vi "Spectral mode.vi"() -> ()   [LabVIEW 2018]
panel:
  in  "Constante de condition\n(Voir l'aide contextuelle)":bool
  out "Data":i32[][](graph)
  out "trigAddress":i32
  in  "Commande tab":T1(tab)
  in  "Area Number to Display":i32
  in  "Reformat":bool
  in  "GAIN":u16(ring) caption="Device Name" items=["High Light", "Best Dynamic Range", "High Sensitivity"]
  in  "ADC":u16(ring) caption="Device Name" items=["20 kHz       ", " 1 MHz       ", "500 kHz Wrap"]
  in  "Number of Areas :":u16=1 min=1 step=1
  in  "Integration time (ms) :":i16=10
  out "Uniques ID":u16(ring) items=["CCD1", "CCD2"]
  in  "Device Name":u16(ring) items=["Synapse CCD (Lateral)", "Synapse_IGA (Axial)"]
  in  "Signal type :":enum16{"TTL Rising Edge", "TTL Falling Edge"}(ring)=enum."TTL Falling Edge"
  in  "Trigger Type :":u16(ring) items=["On Start"=1, "Per Acquisition"=2]
  in  "trigSigTypeString":string
  in  "trigEventString":string
  in  "Enable InputTriggers :":bool
  in  "Number of Cleans":i32=1
  in  "MultiAcqShutterMode":i32(ring)=3 items=["Open For All Spectra"=1, "Open for Each Spectrum"=3]
  in  "Accumulations:":u16=10 min=1 step=1
  in  "Multi Accumulation mode:":bool
  out "Y Pixels:":i32=256
  out "DataSize":i32=1024
  out "X Pixels:":i32=1024
  out "Firmware\nVersion":string="V1.20 CCD_4000"
  out "Acq Time(ms)":u32=3401
  out "Gain Number":i32[](array[numeric])=[10, 11, 12, 13, 8, 2]
  out "ADC Number":i32[](array[numeric])=[0, 1, 2, 3, 4]
  in  "save":bool
  out "initialized ?":bool=TRUE
  in  "Continuous":bool
  in  "CCD Busy":bool
  in  "ShutterOpen":bool=TRUE caption="Shutter enable"
  out "temp graph":dbl(graph)=-134.538067
  in  "Temperature":bool
  out "areas :":i32[][](array[numeric])=[[1], [1], [1], [1024], [256], [1], [256]]
  in  "Acquire":bool
  in  "Setup":bool
  in  "Close":bool=TRUE
  out "indicator":string="Ready !"
  in  "initialize":bool
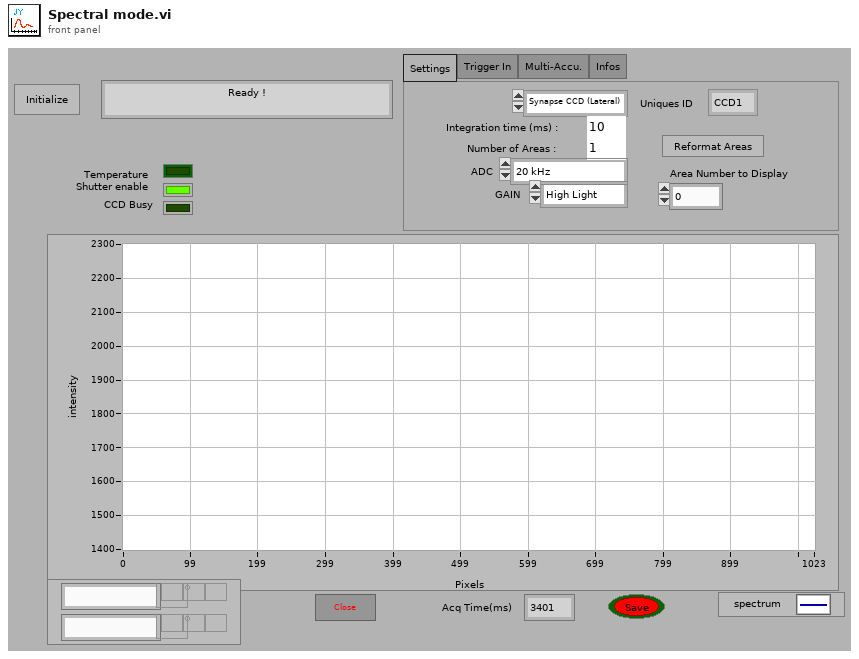
[diagram p1: front panel]
types:
  T1 = enum32{"Settings", "Trigger In", "Multi-Accu.", "Infos"}
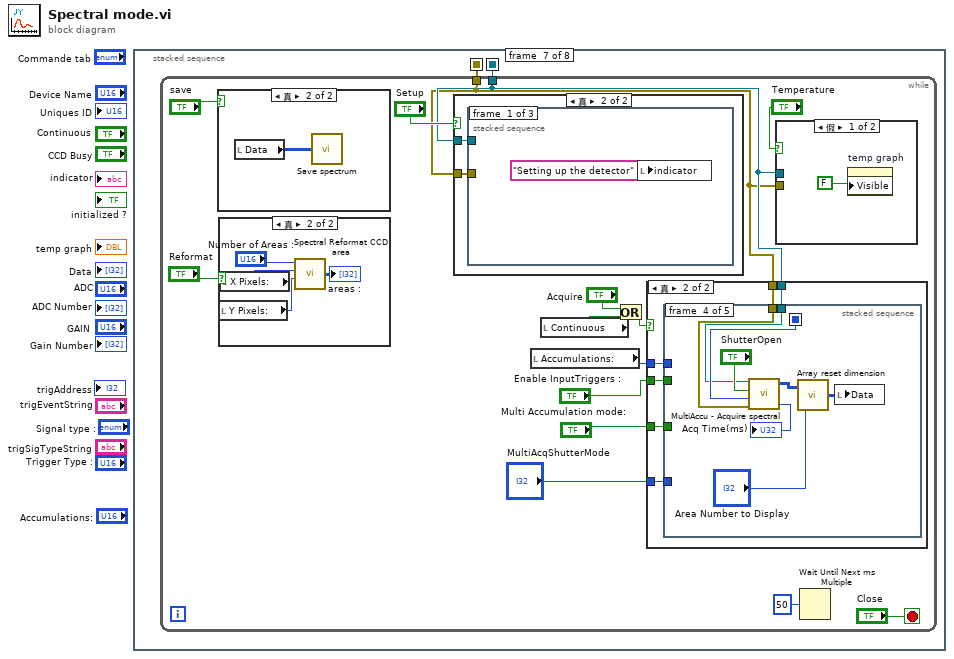
[diagram p0: block diagram]
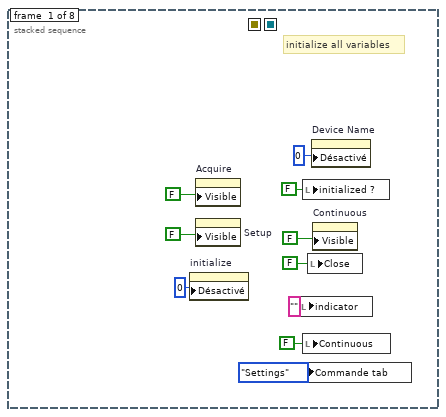
[diagram p2: hidden frame]
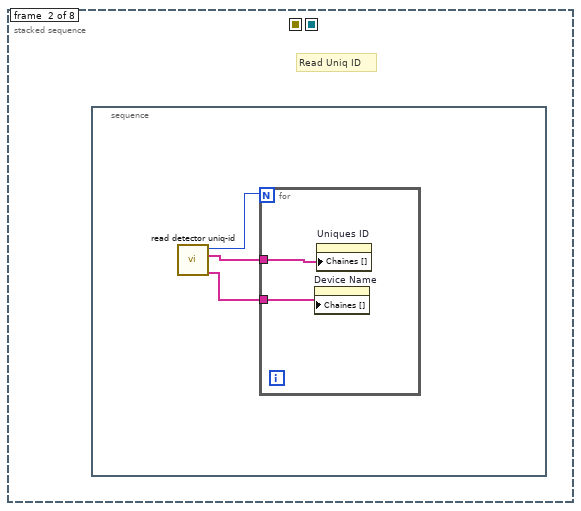
[diagram p3: hidden frame]
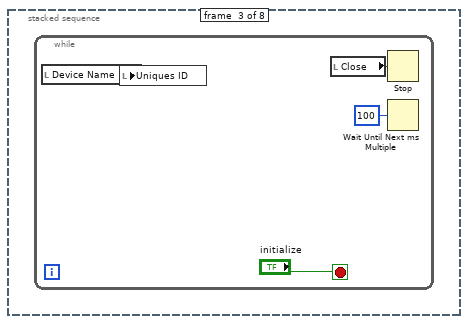
[diagram p4: hidden frame]
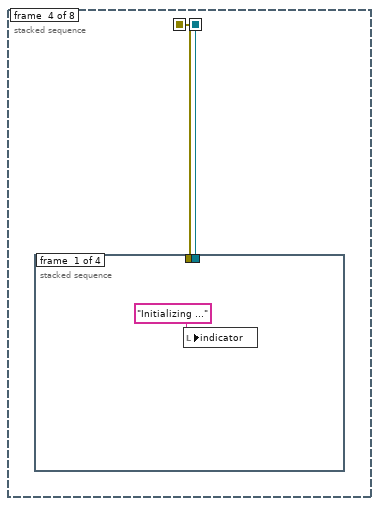
[diagram p5: hidden frame]
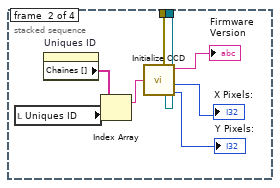
[diagram p6: hidden frame]
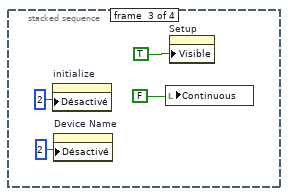
[diagram p7: hidden frame]
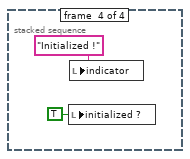
[diagram p8: hidden frame]
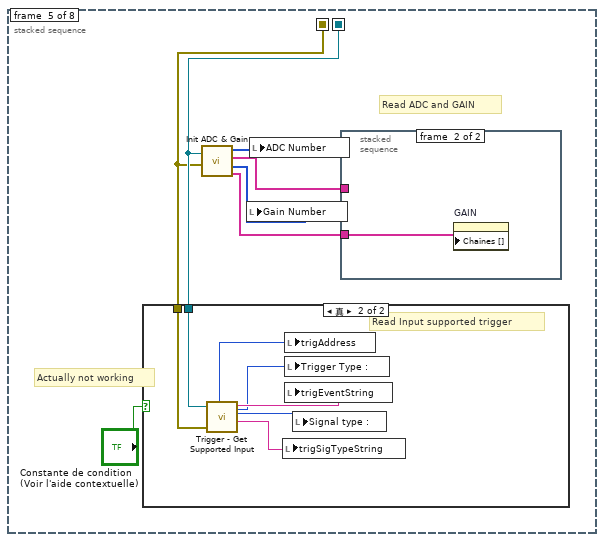
[diagram p9: hidden frame]
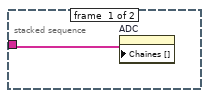
[diagram p11: hidden frame]
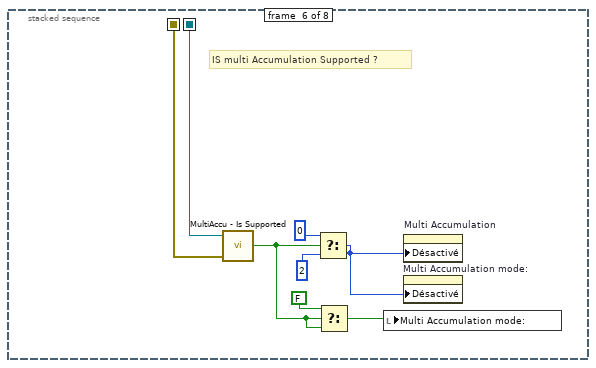
[diagram p12: hidden frame]
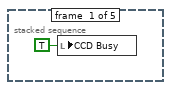
[diagram p15: hidden frame]
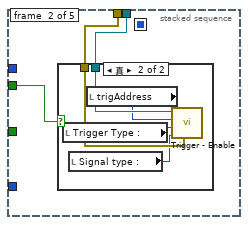
[diagram p16: hidden frame]
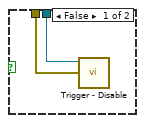
[diagram p17: hidden frame]
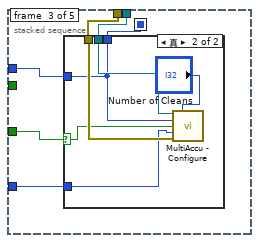
[diagram p18: hidden frame]
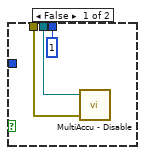
[diagram p19: hidden frame]
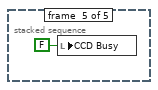
[diagram p20: hidden frame]
diagram:
  n1 = stacked-sequence {
    seq-local: [_ _ _ w21 _ _ _ _] -> [_ _ _ _ w39 w59 w62 w150]
    seq-local: [_ _ _ w20 _ _ _ _] -> [_ _ _ _ w40 w60 w61 w151]
    frame #0 {
      # "initialize all variables"
      n2 = property on="initialize" class="Bool"("Désactivé"=u8 0) -> ()  [unwired: 2 in, 2 out]
      n3 = property on="Acquire" class="Bool"("Visible"=FALSE) -> ()  [unwired: 2 in, 2 out]
      n4 = property on="Setup" class="Bool"("Visible"=FALSE) -> ()  [unwired: 2 in, 2 out]
      n5 = local write "indicator"("" ("indicator")) -> ()
      n6 = local write "Commande tab"(T1."Settings" ("Commande tab")) -> ()
      n7 = local write "initialized ?"(FALSE ("initialized ?")) -> ()
      n8 = local write "Continuous"(FALSE ("Continuous")) -> ()
      n9 = local write "Close"(FALSE ("Close")) -> ()
      n10 = property on="Device Name" class="Ring (严格)"("Désactivé"=u8 0) -> ()  [unwired: 2 in, 2 out]
      n11 = property on="Continuous" class="Bool (严格)"("Visible"=FALSE) -> ()  [unwired: 2 in, 2 out]
    }
    frame #1 {
      # "Read Uniq ID"
      n12 = stacked-sequence {
        frame #0 {
          n13 = call <userlib>:"read detector uniq-id.vi"() -> ("nbr of components"=w13:i32, "UniqueID"=w12:string[], "Name"=w11:string[])  [unwired: 4 out]
          n14 = for {
            N: w13 -> [_]
            tunnel: w12 -> [w15]
            tunnel: w11 -> [w14]
            n15 = property on="Device Name" class="Ring (严格)"("Chaînes []"=w14) -> ()  [unwired: 2 in, 2 out]
            n16 = property on="Uniques ID" class="Ring (严格)"("Chaînes []"=w15) -> ()  [unwired: 2 in, 2 out]
          }
        }
      }
    }
    frame #2 {
      n17 = while {
        stop <- "initialize" stop-if-true
        n18 = local read "Device Name"() -> (w18:u16)
        n19 = local write "Uniques ID"(w18) -> ()
        n20 = local read "Close"() -> (w16:bool)
        n21 = Stop(stop? (T)=w16) -> ()
        n22 = Wait Until Next ms Multiple(millisecond multiple=u32 100 ("n millisecondes")) -> ()  [unwired: 1 out]
      }
    }
    frame #3 {
      n23 = stacked-sequence {
        tunnel: [_ w28 _ _] -> w21
        tunnel: [_ w27 _ _] -> w20
        frame #0 {
          n24 = local write "indicator"("Initializing ..." ("indicator")) -> ()
        }
        frame #1 {
          n25 = local read "Uniques ID"() -> (w25:u16)
          n26 = property on="Uniques ID" class="Ring (严格)"() -> ("Chaînes []"=w26:string[])  [unwired: 2 in, 2 out]
          n27 = Index Array(array=w26, index=w25) -> (element=w24:string)
          n28 = call <userlib>:"Initialize CCD.vi"("Unique id:"=w24) -> ("activeYPixels"=→"Y Pixels:":i32, "JYCCDLib.IJYCCDReqd"=w27:refnum<k7>, "activeXPixels"=→"X Pixels:":i32, "sortie d'erreur"=w28:errorcluster, "FirmwareVersion"=→"Firmware\nVersion":string)  [unwired: 3 out]
        }
        frame #2 {
          n29 = property on="initialize" class="Bool"("Désactivé"=u8 2) -> ()  [unwired: 2 in, 2 out]
          n30 = property on="Device Name" class="Ring (严格)"("Désactivé"=u8 2) -> ()  [unwired: 2 in, 2 out]
          n31 = local write "Continuous"(FALSE ("Continuous")) -> ()
          n32 = property on="Setup" class="Bool"("Visible"=TRUE) -> ()  [unwired: 2 in, 2 out]
        }
        frame #3 {
          n33 = local write "initialized ?"(TRUE ("initialized ?")) -> ()
          n34 = local write "indicator"("Initialized !" ("indicator")) -> ()
        }
      }
    }
    frame #4 {
      # "Actually not working"
      # "Read ADC and GAIN"
      n35 = case shown="真" "Constante de condition\n(Voir l'aide contextuelle)" {
        tunnel: w40 -> [_ w50]
        tunnel: w39 -> [_ w49]
        frame False {
        }
        frame True {
          # "Read Input supported trigger"
          n36 = call <userlib>:"Trigger - Get Supported Input.vi"("JYCCDLib.IJYCCDReqd"=w50, "Error Input"=w49) -> ("trigAddress"=w44:i32, "eventPtr"=w45:i32, "trigEventString"=w48:string, "trigSigType"=w47:i32, "trigSigTypeString"=w46:string)  [unwired: 4 out]
          n37 = local write "trigSigTypeString"(w46) -> ()
          n38 = local write "trigAddress"(w44) -> ()
          n39 = local write "Trigger Type :"(w45) -> ()
          n40 = local write "trigEventString"(w48) -> ()
          n41 = local write "Signal type :"(w47) -> ()
        }
      }
      n42 = call <userlib>:"Init ADC & Gain.vi"("JYCCDLib.IJYCCDReqd"=w40, "input error"=w39) -> ("ADC Number"=w38:i32[], "ADC description"=w43:string[], "Gain Number"=w41:i32[], "Gain description"=w42:string[])
      n43 = local write "Gain Number"(w41) -> ()
      n44 = local write "ADC Number"(w38) -> ()
      n45 = stacked-sequence {
        tunnel: w43 -> [w51 _]
        tunnel: w42 -> [_ w52]
        frame #0 {
          n46 = property on="ADC" class="Ring (严格)"("Chaînes []"=w51) -> ()  [unwired: 2 in, 2 out]
        }
        frame #1 {
          n47 = property on="GAIN" class="Ring (严格)"("Chaînes []"=w52) -> ()  [unwired: 2 in, 2 out]
        }
      }
    }
    frame #5 {
      # "IS multi Accumulation Supported ?"
      n48 = call <userlib>:"MultiAccu - Is Supported.vi"("Error In"=w59, "JYCCDLib.IJYCCDReqd"=w60) -> ("IsOperatingModeSupported"=w53:bool)  [unwired: 3 out]
      n49 = Select(t=0, s=w53, f=2) -> (s? t:f=w56:i32)
      n50 = Select(t=FALSE, s=w53, f=w53) -> (s? t:f=w55:bool)
      n51 = local write "Multi Accumulation mode:"(w55) -> ()
      n52 = property on="Multi Accumulation" class="Bool (严格)"("Désactivé"=w56) -> ()  [unwired: 2 in, 2 out]
      n53 = property on="Multi Accumulation mode:" class="Bool (严格)"("Désactivé"=w56) -> ()  [unwired: 2 in, 2 out]
    }
    frame #6 {
      n54 = while {
        tunnel: w61 -> [w70]
        tunnel: w62 -> [w68]
        stop <- "Close" stop-if-true
        n55 = case shown="真" "save" {
          frame False {
          }
          frame True {
            n56 = local read "Data"() -> (w78:i32[][])
            n57 = call "Save spectrum.vi"("Datas 2"=w78) -> ()  [unwired: 1 out]
          }
        }
        n58 = case shown="真" "Reformat" {
          frame False {
          }
          frame True {
            n59 = local read "Y Pixels:"() -> (w128:i32)
            n60 = local read "X Pixels:"() -> (w130:i32)
            n61 = call <userlib>:"Spectral Reformat CCD area.vi"("Y Pixels:"=w128, "X Pixels:"=w130, "numAreas"="Number of Areas :") -> ("areas :"=→"areas :":i32[][])  [unwired: 3 out]
          }
        }
        n62 = case shown="真" "Setup" {
          tunnel: w68 -> [_ w133]
          tunnel: w70 -> [_ w132]
          frame False {
          }
          frame True {
            n63 = stacked-sequence {
              tunnel: w133 -> [_ w147 _]
              tunnel: w132 -> [_ w144 _]
              frame #0 {
                n64 = local write "indicator"("Setting up the detector" ("indicator")) -> ()
              }
              frame #1 {
                w145 = 1 items=["JYMCD_ACQ_FORMAT_IMAGE", "JYMCD_ACQ_FORMAT_SCAN"] ("Acquisition type")
                n65 = local read "Gain Number"() -> (w139:i32[])
                n66 = local read "GAIN"() -> (w135:u16)
                n67 = local read "ADC Number"() -> (w140:i32[])
                n68 = local read "ADC"() -> (w136:u16)
                n69 = Index Array(array=w139, index=w135) -> (element=w137:i32)
                n70 = Index Array(array=w140, index=w136) -> (element=w138:i32)
                n71 = local read "Number of Areas :"() -> (w142:u16)
                n72 = local read "areas :"() -> (w143:i32[][])
                n73 = call <userlib>:"Setup CCD.vi"("numAreas"=w142, "areas :"=w143, "JYCCDLib.IJYCCDReqd"=w144, "entrée d'erreur (pas d'erreur)"=w147, "Acquisition type"=w145, "Gain"=w137, "Select ADC"=w138, "Integration time(ms)"="Integration time (ms) :") -> ("DataSize"=→"DataSize":i32)  [unwired: 1 out]
              }
              frame #2 {
                w148 = TRUE ("Visible")
                n74 = property on="Continuous" class="Bool (严格)"("Visible"=w148) -> ()  [unwired: 2 in, 2 out]
                n75 = property on="Acquire" class="Bool"("Visible"=w148) -> ()  [unwired: 2 in, 2 out]
                n76 = local write "indicator"("Ready !" ("indicator")) -> ()
              }
            }
          }
        }
        n77 = local read "Accumulations:"() -> (w65:u16)
        n78 = local read "Continuous"() -> (w71:bool)
        n79 = Or(x="Acquire", y=w71) -> (x .or. y?=w67:bool)
        n80 = case shown="真" w67 {
          tunnel: w70 -> [_ w84]
          tunnel: w68 -> [_ w83]
          tunnel: "Enable InputTriggers :" -> [_ w82]
          tunnel: "Multi Accumulation mode:" -> [_ w81]
          tunnel: w65 -> [_ w80]
          tunnel: "MultiAcqShutterMode" -> [_ w79]
          frame False {
          }
          frame True {
            n81 = stacked-sequence {
              seq-local: [_ _ w97 _ _] -> [_ _ _ w116 _]
              tunnel: w84 -> [_ w86 w101 w115 _]
              tunnel: w83 -> [_ w87 w100 w114 _]
              tunnel: w82 -> [_ w88 _ _ _]
              tunnel: w81 -> [_ _ w99 _ _]
              tunnel: w80 -> [_ _ w98 _ _]
              tunnel: w79 -> [_ _ w96 _ _]
              frame #0 {
                n82 = local write "CCD Busy"(TRUE ("CCD Busy")) -> ()
              }
              frame #1 {
                n83 = case shown="真" w88 {
                  tunnel: w87 -> [w89 w95]
                  tunnel: w86 -> [w90 w94]
                  frame False {
                    n84 = call <userlib>:"Trigger - Disable.vi"("Error In"=w89, "JYCCDLib.IJYCCDReqd"=w90) -> ()  [unwired: 6 out]
                  }
                  frame True {
                    n85 = local read "Trigger Type :"() -> (w91:u16)
                    n86 = local read "Signal type :"() -> (w92:enum16{"TTL Rising Edge", "TTL Falling Edge"})
                    n87 = local read "trigAddress"() -> (w93:i32)
                    n88 = call <userlib>:"Trigger - Enable.vi"("Error In"=w95, "sigType"=w92, "event"=w91, "trigAddress"=w93, "JYCCDLib.IJYCCDReqd"=w94) -> ()  [unwired: 3 out]
                  }
                }
              }
              frame #2 {
                n89 = case shown="真" w99 {
                  selector: w99 -> [_ w107]
                  tunnel: w101 -> [w104 w110]
                  tunnel: w100 -> [w103 w109]
                  tunnel: w98 -> [_ w108]
                  tunnel: [u16 1 ("Accumulations:") w108] -> w97
                  tunnel: w96 -> [_ w106]
                  frame False {
                    n90 = call <userlib>:"MultiAccu - Disable.vi"("Error In"=w103, "JYCCDLib.IJYCCDReqd"=w104) -> ()  [unwired: 4 out]
                  }
                  frame True {
                    n91 = call <userlib>:"MultiAccu - Configure.vi"("JYCCDLib.IJYCCDReqd"=w110, "Cleans Before"="Number of Cleans", "Accumulations:"=w108, "MultiAcqHardwareMode"=w107, "MultiAcqShutterMode"=w106, "Error In"=w109) -> ()  [unwired: 1 in, 9 out]
                  }
                }
              }
              frame #3 {
                n92 = call <userlib>:"MultiAccu - Acquire spectral.vi"("error in"=w114, "Accumulations:"=w116, "ShutterOpen"="ShutterOpen", "JYCCDLib.IJYCCDReqd"=w115) -> ("Acq Time(ms)"=→"Acq Time(ms)":u32, "Array Out"=w113:i32[][][])  [unwired: 1 out]
                n93 = call <userlib>:"Array reset dimension.vi"("Area Number"="Area Number to Display", "Array In"=w113) -> ("Array Out"=w112:i32[][])
                n94 = local write "Data"(w112) -> ()
              }
              frame #4 {
                n95 = local write "CCD Busy"(FALSE ("CCD Busy")) -> ()
              }
            }
          }
        }
        n96 = case shown="假" "Temperature" {
          tunnel: w70 -> [_ w122]
          tunnel: w68 -> [_ w121]
          frame False {
            n97 = property on="temp graph" class="WFChart (严格)"("Visible"=FALSE) -> ()  [unwired: 2 in, 2 out]
          }
          frame True {
            n98 = stacked-sequence {
              tunnel: w122 -> [_ w127]
              tunnel: w121 -> [_ w126]
              frame #0 {
                n99 = property on="temp graph" class="WFChart (严格)"("Visible"=TRUE) -> ()  [unwired: 2 in, 2 out]
              }
              frame #1 {
                w125 = u16 0 items=["° Celsius", "Kelvin", "° Farenheit"] ("units")
                n100 = call <userlib>:"read temperature.vi"("entrée d'erreur (pas d'erreur)"=w126, "units"=w125, "JYCCDLib.IJYCCDReqd"=w127) -> ("Current Temperature"=w124:dbl)
                n101 = local write "temp graph"(w124) -> ()
              }
            }
          }
        }
        n102 = Wait Until Next ms Multiple(millisecond multiple=u32 50 ("n millisecondes")) -> ()  [unwired: 1 out]
      }
    }
    frame #7 {
      n103 = Close Reference(reference=w151, error in (no error)=w150) -> ()  [unwired: 1 out]
    }
  }
